vi "ECM_Operating_Mode_Simulator.vi"() -> ()   [LabVIEW 2026]
panel:
  out "ECM Mode History (Mode ID)":dbl(graph)
  out "Vehicle Speed History (km/h)":dbl(graph)
  out "Engine RPM History":dbl(graph)
  out "Vehicle Speed (Km/Hr)":dbl
  out "Engine Speed (RPM)":dbl
  in  "START ECM MODE SIMULATOR":bool
  out "ECM Mode":string
  in  "stop":bool
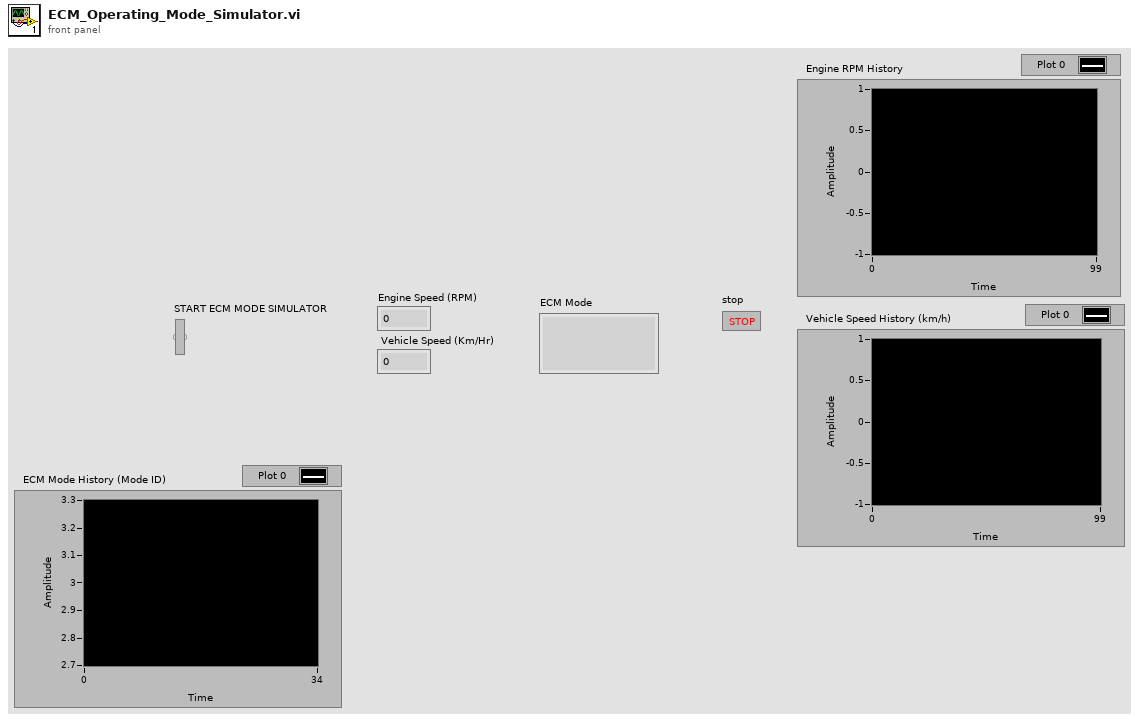
[diagram p1: front panel]
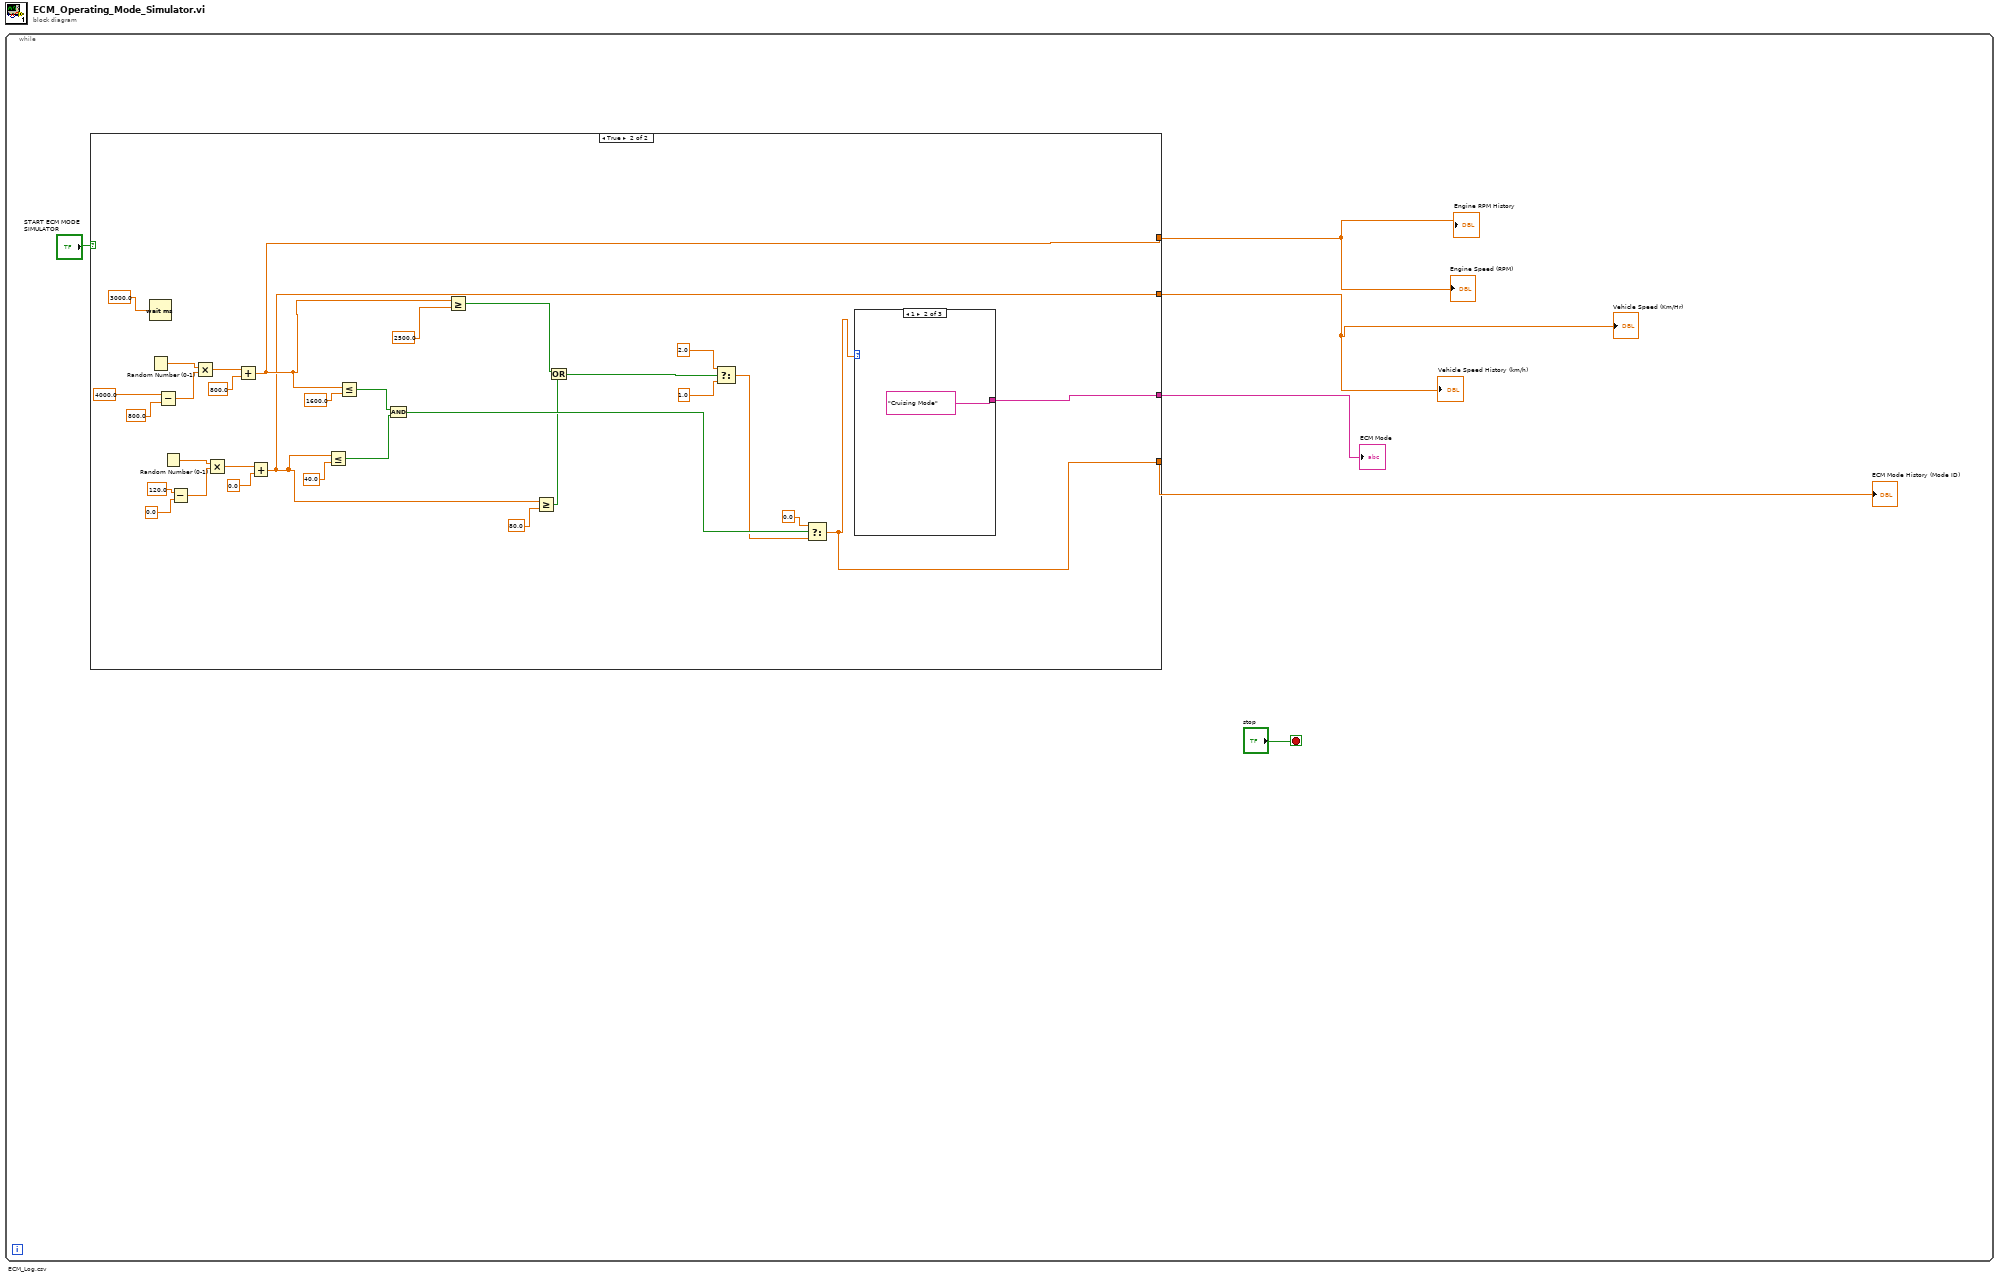
[diagram p0: block diagram]
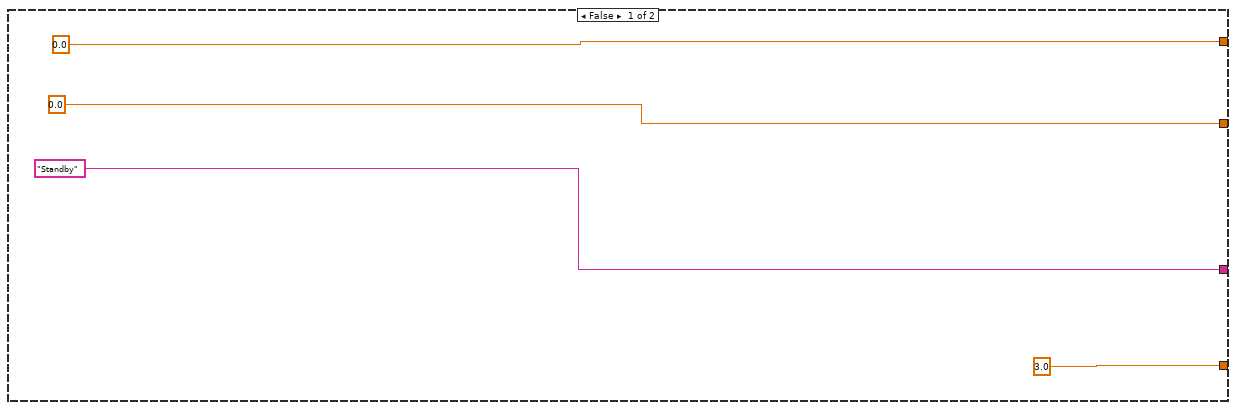
[diagram p2: hidden frame]
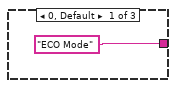
[diagram p3: hidden frame]
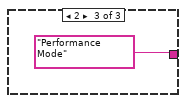
[diagram p4: hidden frame]
diagram:
  # "ECM_Log.csv"
  n1 = while {
    stop <- "stop" stop-if-true
    n2 = case shown="True" "START ECM MODE SIMULATOR" {
      tunnel: [0.0 ("x") w13] -> w3
      tunnel: [0.0 ("x") w11] -> w2
      tunnel: ["Standby" w15] -> w4
      tunnel: [3.0 ("x") w12] -> w1
      frame False {
      }
      frame True {
        n3 = Wait (ms)(milliseconds to wait=3000.0 ("x")) -> ()  [unwired: 1 out]
        n4 = Random Number (0-1)() -> (number: 0 to 1=w30:dbl)
        n5 = Subtract(x=4000.0, y=800.0 ("x")) -> (x-y=w31:dbl)
        n6 = Random Number (0-1)() -> (number: 0 to 1=w32:dbl)
        n7 = Subtract(x=120.0, y=0.0 ("x")) -> (x-y=w33:dbl)
        n8 = Multiply(x=w30, y=w31) -> (x*y=w14:dbl)
        n9 = Multiply(x=w32, y=w33) -> (x*y=w34:dbl)
        n10 = Add(x=w14, y=800.0 ("x")) -> (x+y=w13:dbl)
        n11 = Add(x=w34, y=0.0 ("x")) -> (x+y=w11:dbl)
        n12 = Less Or Equal?(x=w11, y=40.0 ("x")) -> (x <= y?=w35:bool)
        n13 = Less Or Equal?(x=w13, y=1600.0 ("x")) -> (x <= y?=w36:bool)
        n14 = And(x=w36, y=w35) -> (x .and. y?=w40:bool)
        n15 = Greater Or Equal?(x=w13, y=2500.0 ("x")) -> (x >= y?=w38:bool)
        n16 = Greater Or Equal?(x=w11, y=80.0 ("x")) -> (x >= y?=w37:bool)
        n17 = Or(x=w38, y=w37) -> (x .or. y?=w41:bool)
        n18 = Select(t=2.0 ("x"), s=w41, f=1.0 ("x")) -> (s? t:f=w39:dbl)
        n19 = Select(t=0.0 ("x"), s=w40, f=w39) -> (s? t:f=w12:dbl)
        n20 = case shown="1" w12 {
          tunnel: ["ECO Mode" "Cruising Mode" "Performance Mode"] -> w15
          frame 0, Default {
          }
          frame 1 {
          }
          frame 2 {
          }
        }
      }
    }
    "Engine Speed (RPM)" <- w3
    "Vehicle Speed (Km/Hr)" <- w2
    "ECM Mode" <- w4
    "Engine RPM History" <- w3
    "Vehicle Speed History (km/h)" <- w2
    "ECM Mode History (Mode ID)" <- w1
  }
